vi "Main.vi"() -> ()   [LabVIEW 2021]
doc: "This template is for the Queued Message Handler design pattern.\n\nThe Event Handling Loop generates messages based on user interface actions.\n\nThe Message Handling Loop processes messages generated by the Event Handling Loop, or by other messages. The messages are string values, so new messages can be added easily to the Message Cases case structure in the Message Handling Loop. Each message cluster can also provide an optional value for Message Data, which is a variant that can be converted to whatever message-specific data is required."
uses:
  controls/UI Data.ctl
  Main_VI/Control/login_type.ctl
  controls/test_sequence .ctl
  controls/Get_Set.ctl
  Main_VI/Control/Ini.ctl
  Main_VI/Control/Set_Get.ctl
  controls/FGI.ctl
  support/Message Queue/Enqueue Message (Single).vi
  <vilib>/Utility/error.llb/Error Cluster From Error Code.vi
  <vilib>/ErrorRing/Error Ring.xnode
  support/Message Queue/Message Queue.lvlib
  support/User Event - Stop/User Event - Stop.lvlib
  Main_VI/Control/Vi_selection.ctl
panel:
  out "Test Result":string[][](array[string])
  out "Array":bool[](array[boolean])
  out "element":string[][](array[string])
  out "Elapsed Time (s)":dbl
  out "stop":bool
  out "Update timer":bool
  out "reset timer":bool
  out "Result":bool
  in  "Back Button":bool
  out "Tab Control":enum32{" START ", " HOME ", " TEST "}(tab)
  in  "Uncheck":bool
  in  "Check":bool
  out "FAIL":string
  out "TOTAL":string
  out "PASS":string
  out "?":string
  out "?":string
  out "Test Time":string
  out "Applied 4":string
  out "String Indicator":string
  in  "Start Button":bool
  in  "Main Test Status":i32(listbox)=-1
  in  "Report folder":bool
  in  "Exit":bool
  in  "error in (no error)":errorcluster
  out "Display <Replace Me>":string
  in  "Do Something Else <Replace Me>":bool
  # "REV"
  # "TEST TIME"
  # "BARCODE"
  # "TOTAL"
  # "PASS"
  # "FAIL"
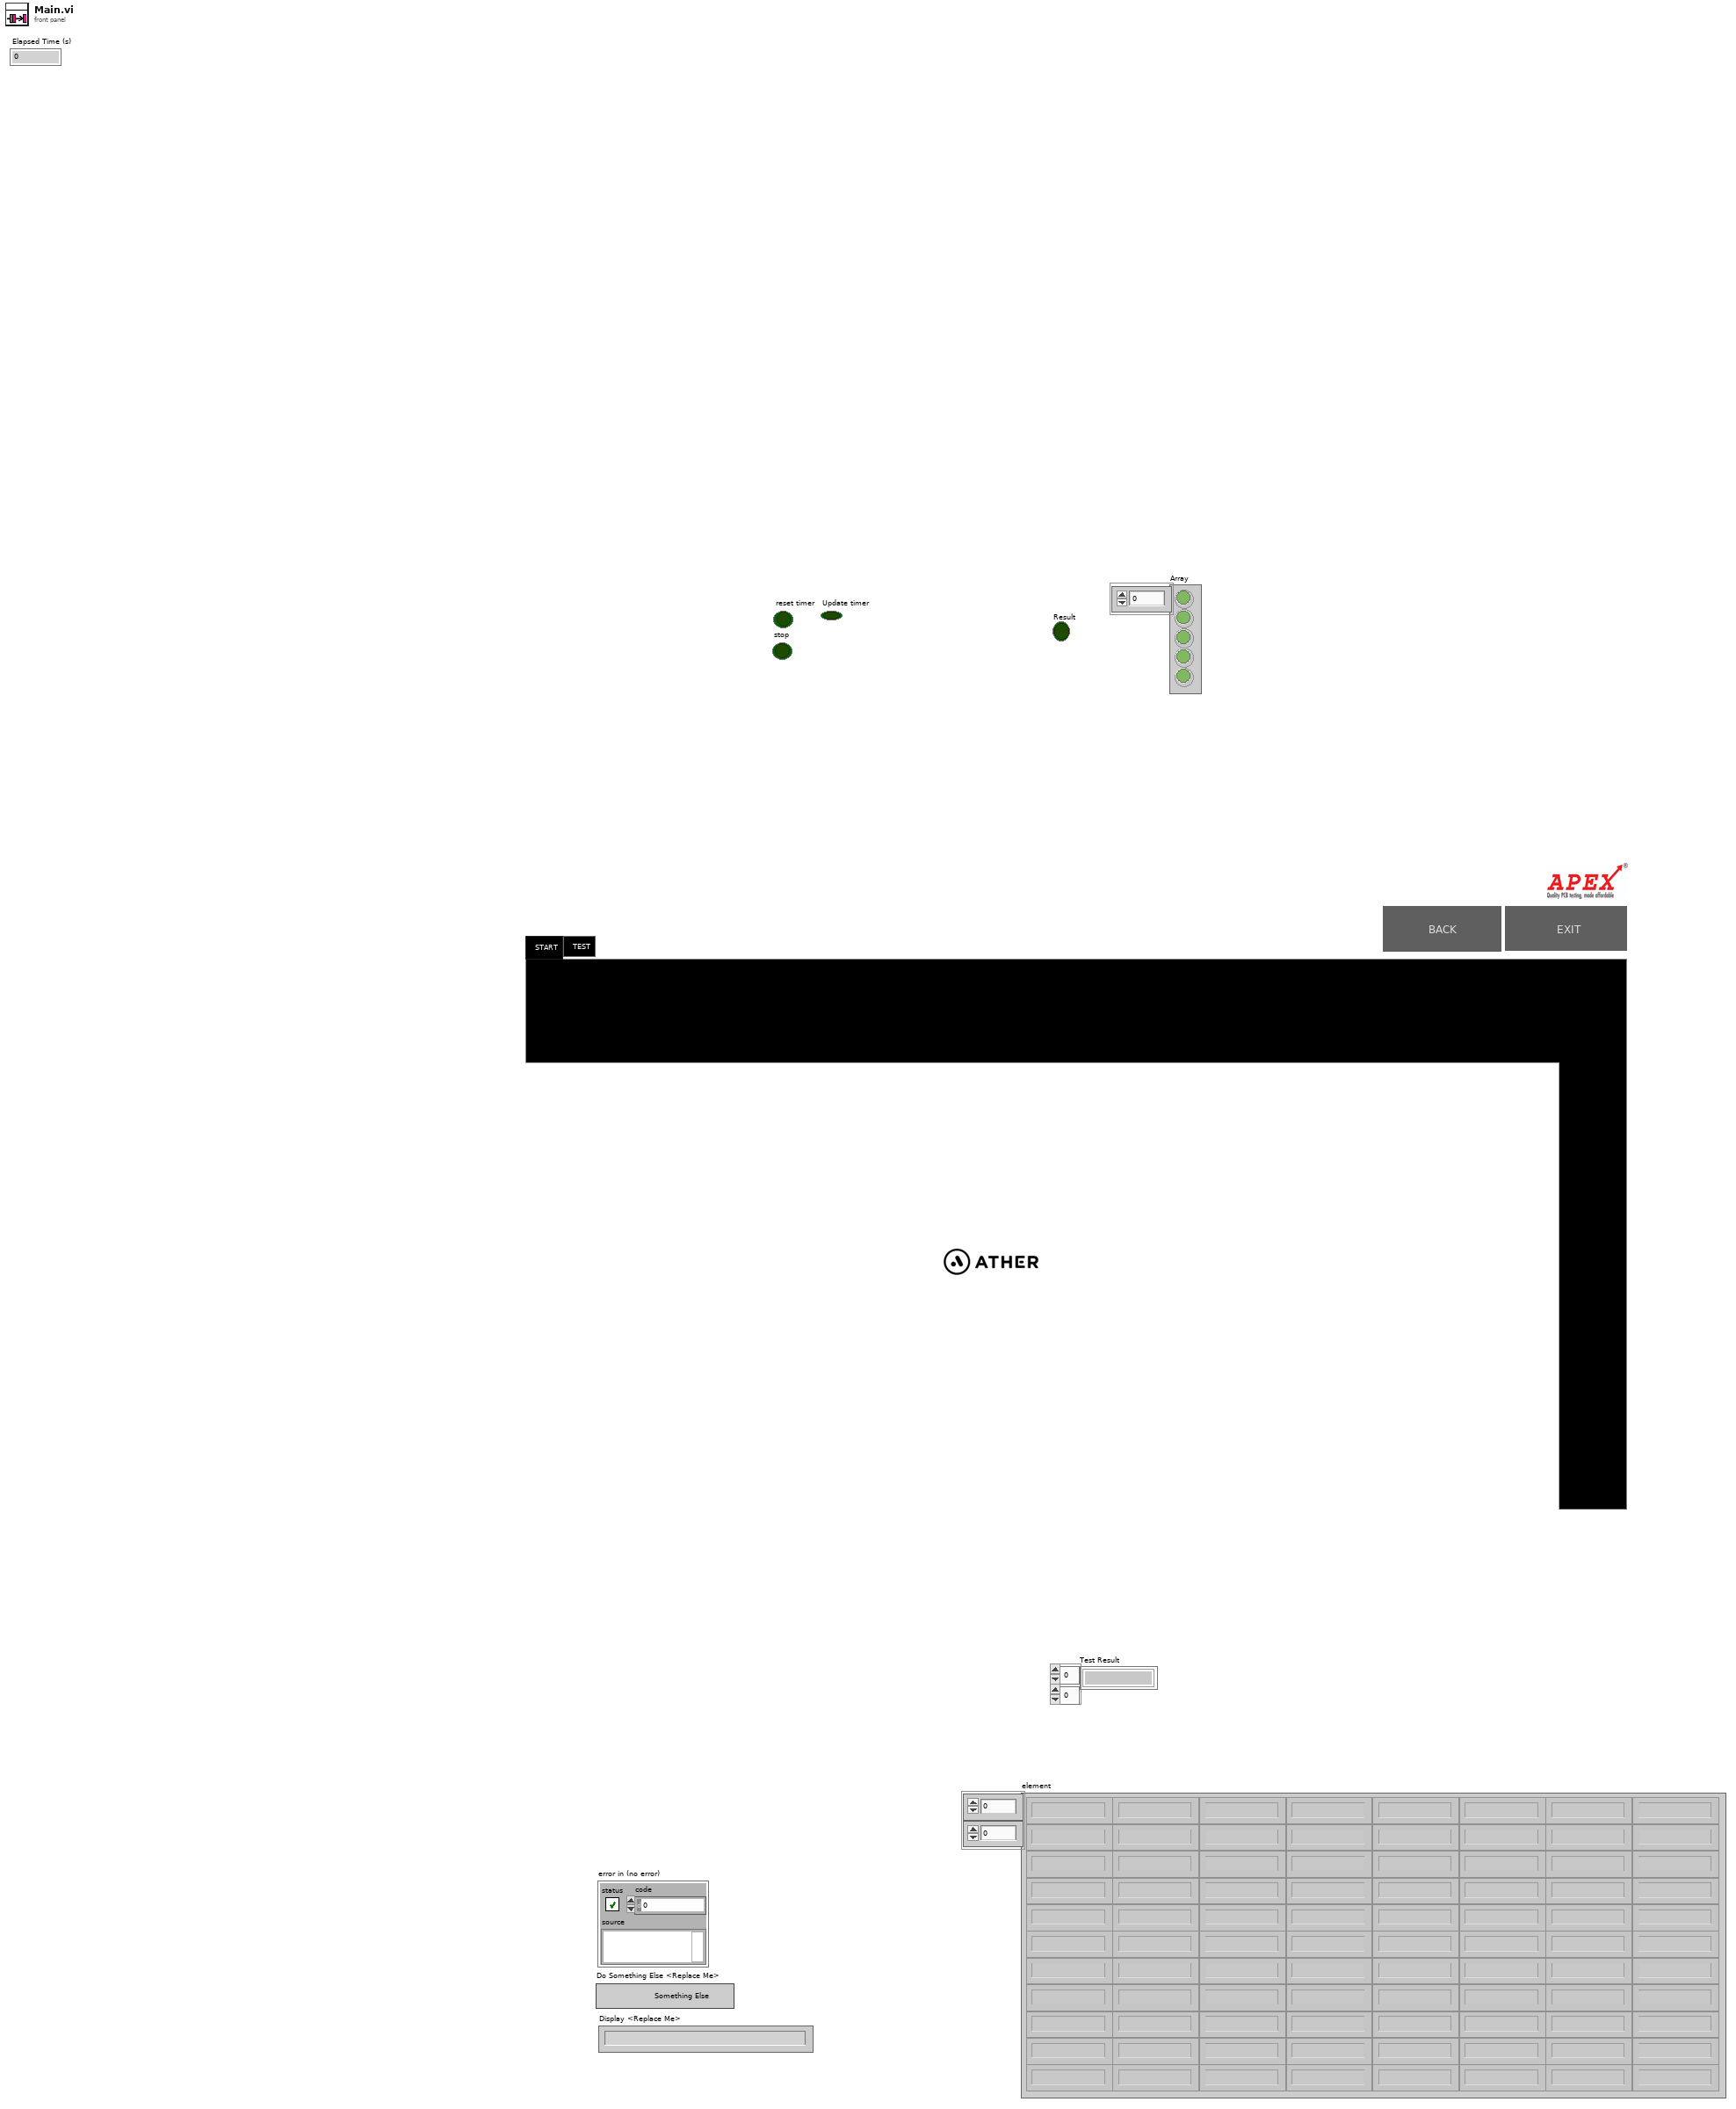
[diagram p1: front panel]
types:
  T1 = typedef "UI Data.ctl" = cluster{"Boolean <Replace Me>":bool, "String <Replace Me>":string, "Numeric <Replace Me>":dbl, "Do Something Ref":refnum<vi>, "Do Something Else Ref":refnum<vi>, "Data Display Ref":refnum<vi>, "Exit Button Ref":refnum<vi>, "Enum":T2, "skip Test  ":bool[]}
  T2 = typedef "login_type.ctl" = enum16{"Operator", "Admin"}
  T3 = typedef "Message Queue.lvlib/All Message Queues.ctl" = cluster{"UI":refnum<queue>}
  T4 = typedef "test_sequence .ctl" = enum16{"Init Devices", "Login", "Option Window", "Idle state", "Check", "Uncheck", "Scan Barcode", "Clear the test Containers", "Init-Pre Test", "Test ", "Result", "Report", "Database", "Update Display", "Confirm Quit", "Error", "Exit"}
  T5 = typedef "LVPoint32TypeDef.ctl" = cluster{"Horizontal":i32, "Vertical":i32}
  T6 = typedef "Ini.ctl" = enum16{"Write", "Read"}
  T7 = enum32{"Invalid", "Standard", "Closed", "Hidden", "Minimized", "Maximized"}
  T8 = typedef "Set_Get.ctl" = enum16{"Set", "Get"}
  T9 = typedef "Vi_selection.ctl" = enum16{"Test Editor", "Option window Vi"}
  T10 = typedef "FGI.ctl" = enum16{"Test Col 1", "Test Col 2"}
  T11 = enum8{"Enabled", "Disabled", "Disabled and Grayed Out"}
  T12 = typedef "Get_Set.ctl" = enum16{"SET", "GET"}
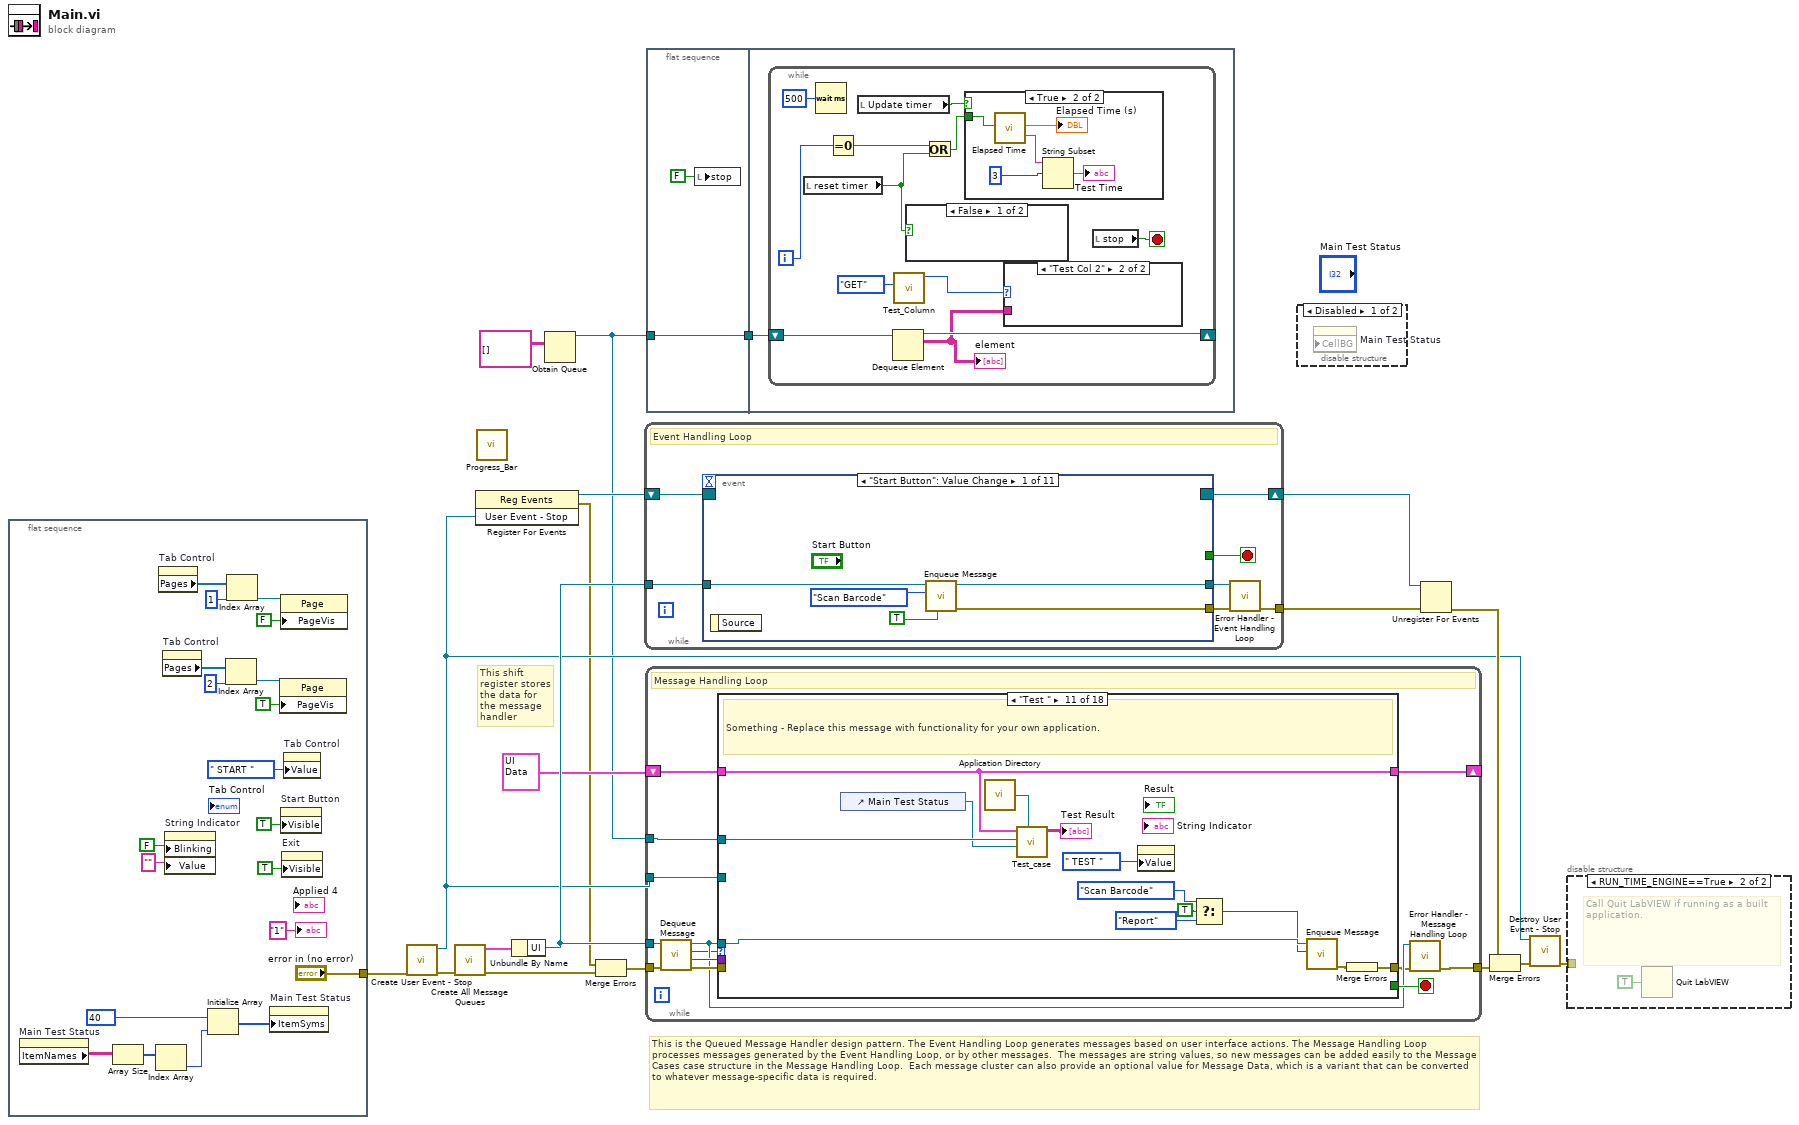
[diagram p0: block diagram]
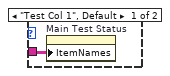
[diagram p3: hidden frame]
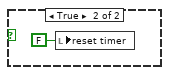
[diagram p4: hidden frame]
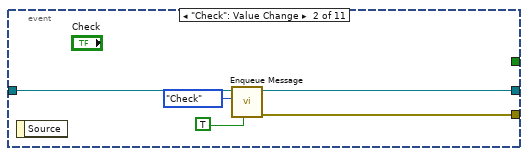
[diagram p7: hidden frame]
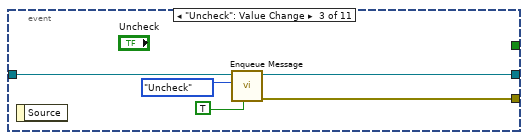
[diagram p8: hidden frame]
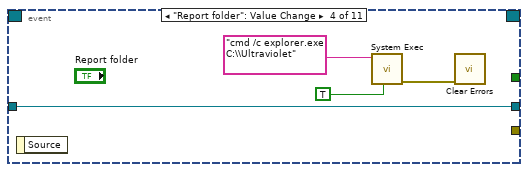
[diagram p9: hidden frame]
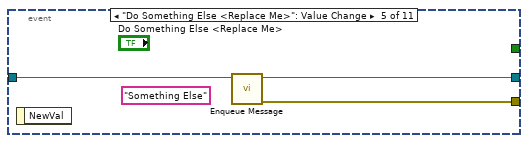
[diagram p10: hidden frame]
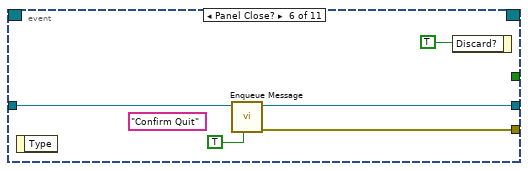
[diagram p11: hidden frame]
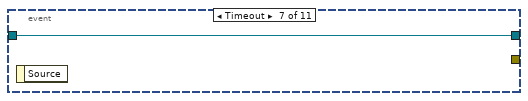
[diagram p12: hidden frame]
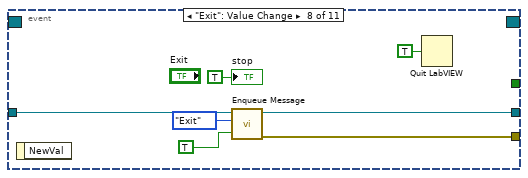
[diagram p13: hidden frame]
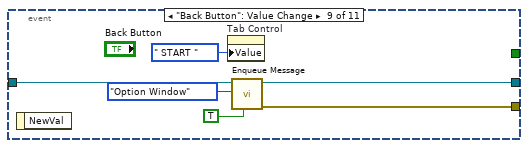
[diagram p14: hidden frame]
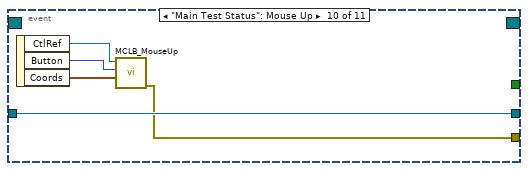
[diagram p15: hidden frame]
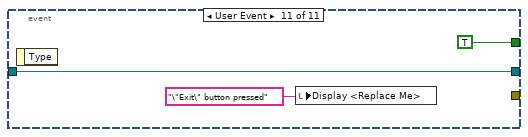
[diagram p16: hidden frame]
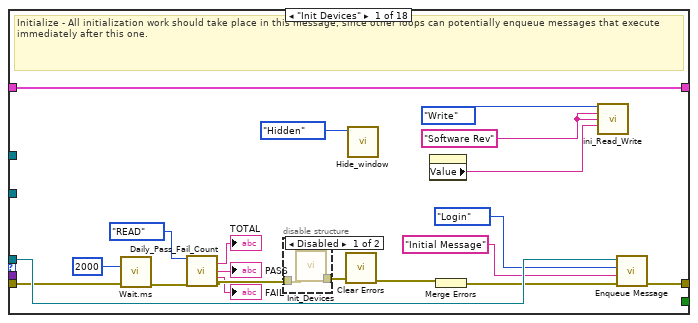
[diagram p17: hidden frame]
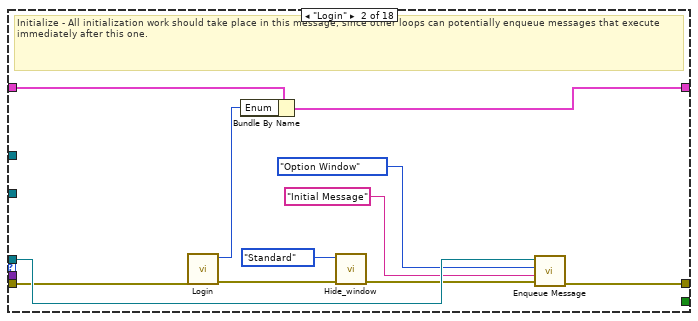
[diagram p19: hidden frame]
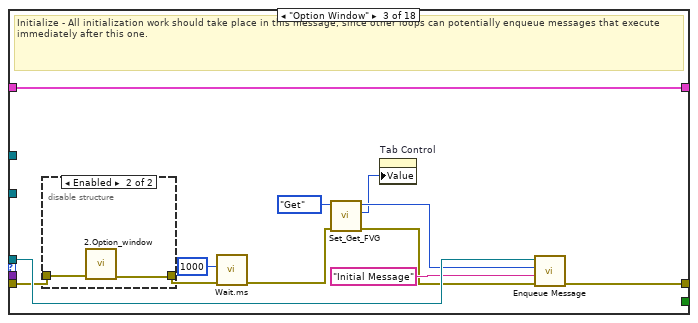
[diagram p20: hidden frame]
diagram:
  # "This is the Queued Message Handler design pattern. The Event Handling Loop generates messages based on user interface actions. The Message Handling Loop processes messages generated by the Event Handling Loop, or by other messages.  The messages are string values, so new messages can be added easily to the Message Cases case structure in the Message Handling Loop.  Each message cluster can also provide an optional value for Message Data, which is a variant that can be converted to whatever message-specific data is required."
  # "This shift register stores the data for the message handler"
  n1 = flat-sequence {
    tunnel: ["error in (no error)"] -> w5
    frame #0 {
      n2 = property on="Main Test Status" class="MCListbox (strict)"() -> ("ItemNames"=w21:string[][])  [unwired: 2 in, 2 out]
      n3 = Array Size(array=w21) -> (size(s)=w22:i32[])
      n4 = Index Array(array=w22) -> (element=w23:i32)  [unwired: 1 in]
      n5 = property on="Tab Control" class="TabCtl (strict)"() -> ("Pages"=w38:refnum<vi>[])  [unwired: 2 in, 2 out]
      n6 = property on="Tab Control" class="TabCtl (strict)"() -> ("Pages"=w32:refnum<vi>[])  [unwired: 2 in, 2 out]
      n7 = property on="String Indicator" class="Str"("Blinking"=FALSE, "Value"="" ("String Indicator")) -> ()  [unwired: 2 in, 2 out]
      n8 = Initialize Array(40, w23) -> (w24:i32[])
      n9 = Index Array(array=w32, index=2) -> (element=w33:refnum<vi>)
      n10 = Index Array(array=w38, index=1) -> (element=w39:refnum<vi>)
      n11 = property on="Main Test Status" class="MCListbox (strict)"("ItemSyms"=w24) -> ()  [unwired: 2 in, 2 out]
      n12 = property class="Page"(reference=w33, "PageVis"=TRUE ("Page Visible")) -> ()  [unwired: 1 in, 2 out]
      n13 = property class="Page"(reference=w39, "PageVis"=FALSE ("Page Visible")) -> ()  [unwired: 1 in, 2 out]
      n14 = property on="Start Button" class="Bool"("Visible"=TRUE) -> ()  [unwired: 2 in, 2 out]
      n15 = property on="Exit" class="Bool"("Visible"=TRUE) -> ()  [unwired: 2 in, 2 out]
      n16 = property on="Tab Control" class="TabCtl (strict)"("Value"=enum32{" START ", " HOME ", " TEST "}." START " ("Tab Control")) -> ()  [unwired: 2 in, 2 out]
      "?" <- "1"
    }
  }
  n17 = call "Create User Event - Stop.vi"("error in (no error)"=w5) -> ("error out"=w15:errorcluster, "User Event - Stop"=w7:refnum<user-event>)  [unwired: 9 in]
  n18 = call "Create All Message Queues.vi"("error in (no error)"=w15) -> ("error out"=w19:errorcluster, "Message Queues out"=w18:T3)  [unwired: 9 in]
  n19 = register-events(w7) -> (reference out=w8:refnum<event-registration>, error out=w4:errorcluster)  [unwired: 2 in]
  n20 = call "Progress_Bar.vi"() -> ()  [unwired: 11 in, 1 out]
  n21 = Unbundle By Name(w18) -> ("UI"=w16:refnum<queue>)
  n22 = Obtain Queue(element data type=string[][] [] ("Test status item names")) -> (queue out=w1:refnum<queue>)  [unwired: 4 in, 2 out]
  n23 = Merge Errors(w4, w19) -> (w6:errorcluster)
  n24 = while {
    tunnel: w16 -> [w46]
    shift-right: [w44] -> w12
    shift-left: w8 -> [w45]
    tunnel: [w40] -> w9
    stop <- w42 stop-if-true
    # "Event Handling Loop"
    n25 = event shown="[0] \"Start Button\": Value Change" {
      selector: w45 -> [_ _ _ _ _ _ _ _ _ _ _]
      dyn-events: [_ _ _ _ _ _ _ _ _ _ _] -> w44
      timeout: _ -> [_ _ _ _ _ _ _ _ _ _ _]
      tunnel: [_ _ _ _ _ _ _ _ _ _ TRUE ("Discard?")] -> w42
      tunnel: w46 -> [w51 w56 w61 w65 w68 w72 w74 w81 w87 w92 w95]
      tunnel: [w49 w54 w59 _ w66 w71 _ w80 w86 w91 _] -> w43
      tunnel: [w50 w55 w60 w65 w67 w70 w74 w79 w85 w92 w95] -> w41
      event "Start Button": Value Change {
        n26 = event-data() -> ()  [unwired: 1 in, 1 out]
        n27 = call-poly "Enqueue Message.vi"("Priority Message? (F)"=TRUE, "Message"=test_sequence_."Scan Barcode", "Message Queue"=w51) -> ("error out"=w49:errorcluster, "dup Message Queue"=w50:refnum<queue>)  [unwired: 7 in]
      }
      event "Check": Value Change {
        n28 = event-data() -> ()  [unwired: 1 in, 1 out]
        n29 = call-poly "Enqueue Message.vi"("Priority Message? (F)"=TRUE, "Message"=test_sequence_."Check", "Message Queue"=w56) -> ("error out"=w54:errorcluster, "dup Message Queue"=w55:refnum<queue>)  [unwired: 7 in]
      }
      event "Uncheck": Value Change {
        n30 = event-data() -> ()  [unwired: 1 in, 1 out]
        n31 = call-poly "Enqueue Message.vi"("Priority Message? (F)"=TRUE, "Message"=test_sequence_."Uncheck", "Message Queue"=w61) -> ("error out"=w59:errorcluster, "dup Message Queue"=w60:refnum<queue>)  [unwired: 7 in]
      }
      event "Report folder": Value Change {
        n32 = event-data() -> ()  [unwired: 1 in, 1 out]
        n33 = call <vilib>:"System Exec.vi"("run minimized? (F)"=TRUE, "command line"="cmd /c explorer.exe C:\\Ultraviolet") -> ("error out"=w62:errorcluster)  [unwired: 6 in, 3 out]
        n34 = call <vilib>:"Clear Errors.vi"("error in (no error)"=w62) -> ()  [unwired: 5 in, 2 out]
      }
      event "Do Something Else <Replace Me>": Value Change {
        (unwired) "Something Else" ("Message")
        n35 = event-data() -> ()  [unwired: 1 in, 1 out]
        n36 = call-poly "Enqueue Message.vi"("Message Queue"=w68) -> ("error out"=w66:errorcluster, "dup Message Queue"=w67:refnum<queue>)  [unwired: 9 in]
      }
      event Panel Close? {
        (unwired) "Confirm Quit" ("Message")
        n37 = event-data() -> ()  [unwired: 1 in, 1 out]
        n38 = call-poly "Enqueue Message.vi"("Priority Message? (F)"=TRUE, "Message Queue"=w72) -> ("error out"=w71:errorcluster, "dup Message Queue"=w70:refnum<queue>)  [unwired: 8 in]
        n39 = event-data("Discard?"=TRUE) -> ()  [unwired: 1 in, 1 out]
      }
      event Timeout {
        n40 = event-data() -> ()  [unwired: 1 in, 1 out]
      }
      event "Exit": Value Change {
        n41 = event-data() -> ()  [unwired: 1 in, 1 out]
        n42 = call-poly "Enqueue Message.vi"("Priority Message? (F)"=TRUE, "Message"=test_sequence_."Exit", "Message Queue"=w81) -> ("error out"=w80:errorcluster, "dup Message Queue"=w79:refnum<queue>)  [unwired: 7 in]
        n43 = Quit LabVIEW(quit? (T)=TRUE) -> ()
        "stop" <- TRUE ("stop")
      }
      event "Back Button": Value Change {
        n44 = event-data() -> ()  [unwired: 1 in, 1 out]
        n45 = property on="Tab Control" class="TabCtl (strict)"("Value"=enum32{" START ", " HOME ", " TEST "}." START " ("Tab Control")) -> ()  [unwired: 2 in, 2 out]
        n46 = call-poly "Enqueue Message.vi"("Priority Message? (F)"=TRUE, "Message"=test_sequence_."Option Window", "Message Queue"=w87) -> ("error out"=w86:errorcluster, "dup Message Queue"=w85:refnum<queue>)  [unwired: 7 in]
      }
      event "Main Test Status": Mouse Up {
        n47 = event-data() -> ("CtlRef"=w88:refnum<vi>, "Button"=w89:u16, "Coords"=w90:T5)  [unwired: 1 in]
        n48 = call "MCLB_MouseUp.vi"("Coords"=w90, "Button"=w89, "CtlRef"=w88) -> ("error out"=w91:errorcluster)  [unwired: 8 in]
      }
      event User Event {
        n49 = event-data() -> ()  [unwired: 1 in, 1 out]
        n50 = local write "Display <Replace Me>"("\"Exit\" button pressed" ("VI Stopped")) -> ()
      }
    }
    n51 = call "Error Handler - Event Handling Loop.vi"("error in (no error)"=w43, "Message Queue"=w41) -> ("dup error in"=w40:errorcluster)  [unwired: 8 in, 1 out]
  }
  n52 = while {
    tunnel: w16 -> [w101]
    shift-right: [w107] -> _
    shift-left: T1 {"Boolean <Replace Me>"=FALSE, "String <Replace Me>"="", "Numeric <Replace Me>"=0.0, "Do Something Ref"=refnum, "Do Something Else Ref"=refnum, "Data Display Ref"=refnum, "Exit Button Ref"=refnum, "Enum"=enum."Admin", "skip Test  "=[]} ("Data Cluster") -> [w108]
    tunnel: w7 -> [w105]
    tunnel: w6 -> [w104]
    tunnel: [w99] -> w17
    tunnel: w1 -> [w96]
    stop <- w106 stop-if-true
    # "Message Handling Loop"
    n53 = call "Dequeue Message.vi"("error in (no error)"=w104, "Message Queue"=w101) -> ("error out"=w103:errorcluster, "Message Data"=w102:variant, "Message"=w97:T4, "dup Message Queue"=w100:refnum<queue>)  [unwired: 6 in]
    n54 = case "Message Cases" shown="\"Test \"" w97 {
      selector: w97 -> [_ _ _ _ _ _ _ _ _ _ _ _ _ _ _ _ _ w344]
      tunnel: w100 -> [w127 w141 w153 _ _ w179 w189 w219 w245 w252 w272 w290 w302 w312 _ w327 w343 _]
      tunnel: w103 -> [w111 w138 w150 w165 w177 w181 w191 w213 w242 w256 _ w288 w298 w309 w324 w331 w336 _]
      tunnel: [w128 w142 w154 w166 w177 w180 w190 w221 w247 w260 w274 w292 w304 w314 w318 w329 w339 w345] -> w98
      tunnel: w108 -> [w125 w137 w151 w167 w176 w187 w197 w200 w248 w261 w265 w293 w305 w315 w323 w330 w342 w346]
      tunnel: [w125 w136 w151 w167 w176 w187 w197 w198 w248 w261 w265 w293 w305 w315 w323 w330 w342 w346] -> w107
      tunnel: [_ _ _ _ _ _ _ _ _ _ _ _ _ _ _ _ TRUE _] -> w106
      tunnel: w102 -> [_ _ _ w164 _ _ _ _ _ _ _ _ _ _ w322 _ w333 _]
      tunnel: w105 -> [_ _ _ _ _ _ _ _ _ _ _ _ _ _ _ _ w338 _]
      tunnel: w96 -> [_ _ _ _ _ _ _ _ _ _ w266 _ _ _ _ _ _ _]
      frame "Init Devices" {
        w118 = "Software Rev" ("Write Section")
        # "Initialize - All initialization work should take place in this message, since other loops can potentially enqueue messages that execute immediately after this one."
        n55 = call "Wait.ms.vi"("error in"=w111, "milliseconds to wait"=u32 2000) -> ("error out"=w110:errorcluster)  [unwired: 9 in]
        n56 = call "Daily_Pass_Fail_Count.vi"("Action"=enum16{"READ", "WRITE"}."READ", "error in"=w110) -> ("TOTAL"=→"TOTAL":string, "PASS"=→"PASS":string, "FAIL"=→"FAIL":string, "error out"=w116:errorcluster)  [unwired: 8 in, 2 out]
        n57 = disable-structure shown="Disabled" {
          disable-tunnel: [w130 w131] -> w124
          disable-tunnel: w116 -> [w129 w131]
          frame Disabled {
            n58 = call "Init_Devices.vi"("error in"=w129) -> ("error out"=w130:errorcluster)  [unwired: 9 in, 1 out]
          }
          frame Enabled {
          }
        }
        n59 = call <vilib>:"Clear Errors.vi"("error in (no error)"=w124) -> ("error out"=w122:errorcluster)  [unwired: 5 in, 1 out]
        n60 = call "Hide_window.vi"("State"=T7."Hidden") -> ()  [unwired: 10 in, 1 out]
        n61 = property class="Str"() -> ("Value"=w117:string)  [unwired: 2 in, 2 out]
        n62 = Merge Errors(w122) -> (w123:errorcluster)
        n63 = call "ini_Read_Write.vi"(0:Ini."Write", "Write Section"=w118, "Write key"=w118, "Write"=w117) -> ()  [unwired: 10 in, 2 out]
        n64 = call-poly "Enqueue Message.vi"("error in (no error)"=w123, "Message Data"="Initial Message" ("Initial Message"), "Message"=test_sequence_."Login", "Message Queue"=w127) -> ("error out"=w128:errorcluster)  [unwired: 6 in, 1 out]
      }
      frame "Login" {
        # "Initialize - All initialization work should take place in this message, since other loops can potentially enqueue messages that execute immediately after this one."
        n65 = call "Login.vi"("error in (no error) 3"=w138) -> ("error in (no error) 4"=w134:errorcluster, "Enum"=w132:T2)  [unwired: 9 in]
        n66 = Bundle By Name(cluster=w137, "Enum"=w132) -> (w136:T1)
        n67 = call "Hide_window.vi"("error in (no error)"=w134, "State"=T7."Standard") -> ("error out"=w133:errorcluster)  [unwired: 9 in]
        n68 = call-poly "Enqueue Message.vi"("error in (no error)"=w133, "Message Data"="Initial Message" ("Initial Message"), "Message"=test_sequence_."Option Window", "Message Queue"=w141) -> ("error out"=w142:errorcluster)  [unwired: 6 in, 1 out]
      }
      frame "Option Window" {
        # "Initialize - All initialization work should take place in this message, since other loops can potentially enqueue messages that execute immediately after this one."
        n69 = disable-structure shown="Enabled" {
          disable-tunnel: w150 -> [w157 w159]
          disable-tunnel: [w156 w158] -> w149
          frame Disabled {
            n70 = call "3.Open_Vi.vi"("error in (no error)"=w157, "VI Selection"=Vi_selection."Option window Vi") -> ("error out"=w156:errorcluster)  [unwired: 9 in]
          }
          frame Enabled {
            n71 = call "2.Option_window.vi"("error in (no error) 2"=w159) -> ("error in (no error) 3"=w158:errorcluster)  [unwired: 10 in]
          }
        }
        n72 = call "Wait.ms.vi"("error in"=w149, "milliseconds to wait"=u32 1000) -> ("error out"=w145:errorcluster)  [unwired: 9 in]
        n73 = call "Set_Get_FVG.vi"("error out"=w145, "Enum"=Set_Get."Get") -> ("error out 2"=w144:errorcluster, "Tab Control 2"=w143:enum32{" START ", " HOME ", " TEST "}, "Message 2"=w146:T4)  [unwired: 7 in]
        n74 = property on="Tab Control" class="TabCtl (strict)"("Value"=w143) -> ()  [unwired: 2 in, 2 out]
        n75 = call-poly "Enqueue Message.vi"("error in (no error)"=w144, "Message Data"="Initial Message" ("Initial Message"), "Message"=w146, "Message Queue"=w153) -> ("error out"=w154:errorcluster)  [unwired: 6 in, 1 out]
      }
      frame "Update Display" {
        w161 = T11."Enabled" ("Disabled")
        # "Update Display - Convert the message data to a string to display in the Data Display indicator."
        n76 = disable-structure shown="Enabled" {
          disable-tunnel: w165 -> [w172 w173]
          disable-tunnel: w164 -> [w171 _]
          disable-tunnel: [w169 w173] -> w160
          frame Disabled {
            n77 = Variant To Data(error in=w172, type="", Variant=w171) -> (data=→"Display <Replace Me>":string, error out=w169:errorcluster)
          }
          frame Enabled {
          }
        }
        n78 = property class="Str"("Value"="") -> ()  [unwired: 2 in, 2 out]
        n79 = property on="Applied 4" class="Str"("Value"="" ("Applied 4")) -> ()  [unwired: 2 in, 2 out]
        n80 = property on="Start Button" class="Bool"("DisabledEnum"=w161) -> ()  [unwired: 2 in, 2 out]
        n81 = property on="Back Button" class="Bool"("DisabledEnum"=w161) -> ()  [unwired: 2 in, 2 out]
        n82 = property on="Exit" class="Bool"("DisabledEnum"=w161) -> ()  [unwired: 2 in, 2 out]
        n83 = Merge Errors(w160) -> (w166:errorcluster)
      }
      frame "Idle state" {
        w174 = T11."Enabled" ("Disabled")
        n84 = property on="Applied 4" class="Str"("Value"="" ("Applied 4")) -> ()  [unwired: 2 in, 2 out]
        n85 = property on="Start Button" class="Bool"("DisabledEnum"=w174) -> ()  [unwired: 2 in, 2 out]
        n86 = property on="Back Button" class="Bool"("DisabledEnum"=w174) -> ()  [unwired: 2 in, 2 out]
        n87 = property on="Exit" class="Bool"("DisabledEnum"=w174) -> ()  [unwired: 2 in, 2 out]
      }
      frame "Uncheck" {
        n88 = property on="Main Test Status" class="MCListbox (strict)"() -> ("ItemNames"=w185:string[][])  [unwired: 2 in, 2 out]
        n89 = Array Size(array=w185) -> (size(s)=w184:i32[])
        n90 = Index Array(array=w184) -> (element=w183:i32)  [unwired: 1 in]
        n91 = Initialize Array(39, w183) -> (w182:i32[])
        n92 = property on="Main Test Status" class="MCListbox (strict)"("ItemSyms"=w182) -> ()  [unwired: 2 in, 2 out]
        n93 = call-poly "Enqueue Message.vi"("error in (no error)"=w181, "Message"=test_sequence_."Idle state", "Message Queue"=w179) -> ("error out"=w180:errorcluster)  [unwired: 7 in, 1 out]
      }
      frame "Check" {
        n94 = property on="Main Test Status" class="MCListbox (strict)"() -> ("ItemNames"=w195:string[][])  [unwired: 2 in, 2 out]
        n95 = Array Size(array=w195) -> (size(s)=w194:i32[])
        n96 = Index Array(array=w194) -> (element=w193:i32)  [unwired: 1 in]
        n97 = Initialize Array(40, w193) -> (w192:i32[])
        n98 = property on="Main Test Status" class="MCListbox (strict)"("ItemSyms"=w192) -> ()  [unwired: 2 in, 2 out]
        n99 = call-poly "Enqueue Message.vi"("error in (no error)"=w191, "Message"=test_sequence_."Idle state", "Message Queue"=w189) -> ("error out"=w190:errorcluster)  [unwired: 7 in, 1 out]
      }
      frame "Scan Barcode" {
        # "Something - Replace this message with functionality for your own application."
        n100 = property class="Str"(error in=w213, "Value"="") -> (error out=w212:errorcluster)  [unwired: 1 in, 1 out]
        n101 = call "MSG display box two buttons.vi"("error in"=w212, "input string"="Place the DUT , Close The Top Gate and Press OK or Prees ENTER key\n\nThen DO NOT TOUCH FIXTURE") -> ("error out"=w208:errorcluster, "Panel close"=w210:bool)  [unwired: 7 in, 1 out]
        n102 = property on="Tab Control" class="TabCtl (strict)"("Value"=enum32{" START ", " HOME ", " TEST "}." TEST " ("Tab Control")) -> ()  [unwired: 2 in, 2 out]
        n103 = case shown="False" w210 {
          tunnel: w208 -> [w226 w239]
          tunnel: [w228 w239] -> w203
          tunnel: [w227 TRUE ("Time has Elapsed")] -> w211
          frame False {
            n104 = case shown="False" FALSE {
              tunnel: [w231 _] -> w228
              tunnel: [w230 FALSE ("Time has Elapsed")] -> w227
              tunnel: w226 -> [w229 _]
              frame False {
                n105 = disable-structure shown="Disabled" {
                  disable-tunnel: [w235 _] -> w231
                  disable-tunnel: [w234 _] -> w230
                  disable-tunnel: w229 -> [w232 _]
                  frame Disabled {
                    n106 = call "Barcode user prompt.vi"("error in"=w232) -> ("error out"=w235:errorcluster, "Time has Elapsed"=w234:bool, "BARCODE"=→"?":string)  [unwired: 8 in]
                  }
                  frame Enabled {
                  }
                }
              }
              frame True {
                n107 = One Button Dialog(message="              INTERLOCK OPEN \nClose the top gate and press start") -> ()  [unwired: 1 in, 1 out]
              }
            }
          }
          frame True {
          }
        }
        n108 = property on="Main Test Status" class="MCListbox (strict)"() -> ("ItemSyms"=w201:i32[])  [unwired: 2 in, 2 out]
        n109 = property on="Applied 4" class="Str"(error in=w208, "Value"="SCANNING BARCODE" ("Applied 4")) -> ()  [unwired: 1 in, 2 out]
        n110 = for {
          tunnel: w201 -> [w224] mode=indexing
          tunnel: [w222] -> w199 mode=indexing
          n111 = Equal?(x=w224, y=40) -> (x = y?=w222:bool)
        }
        "Array" <- w199
        n112 = Compound Arithmetic op=OR(w211, w210) -> (w209:bool)
        n113 = Bundle By Name(cluster=w200, "skip Test"=w199) -> (w198:T1)
        n114 = Select(t=test_sequence_."Idle state", s=w209, f=test_sequence_."Clear the test Containers" ("Message")) -> (s? t:f=w215:T4)
        n115 = call "Start_Time.vi"("error in (no error)"=w203) -> ("error in (no error) 3"=w204:errorcluster)  [unwired: 10 in]
        n116 = call-poly "Enqueue Message.vi"("error in (no error)"=w204, "Message"=w215, "Message Queue"=w219) -> ("error out"=w220:errorcluster)  [unwired: 7 in, 1 out]
        n117 = property on="String Indicator" class="Str"("Blinking"=FALSE, "Value"="" ("String Indicator")) -> ()  [unwired: 2 in, 2 out]
        n118 = Merge Errors(w220) -> (w221:errorcluster)
      }
      frame "Clear the test Containers" {
        w241 = TRUE ("reset timer")
        w240 = T11."Disabled and Grayed Out" ("Disabled")
        # "Something - Replace this message with functionality for your own application."
        n119 = property on="Tab Control" class="TabCtl (strict)"("Value"=enum32{" START ", " HOME ", " TEST "}." TEST " ("Tab Control")) -> ()  [unwired: 2 in, 2 out]
        n120 = call-poly "Enqueue Message.vi"("error in (no error)"=w242, "Message"=test_sequence_."Init-Pre Test", "Message Queue"=w245) -> ("error out"=w246:errorcluster)  [unwired: 7 in, 1 out]
        n121 = property on="Start Button" class="Bool"("DisabledEnum"=w240) -> ()  [unwired: 2 in, 2 out]
        n122 = property on="Exit" class="Bool"("DisabledEnum"=w240) -> ()  [unwired: 2 in, 2 out]
        n123 = property on="Back Button" class="Bool"("DisabledEnum"=w240) -> ()  [unwired: 2 in, 2 out]
        n124 = Merge Errors(w246) -> (w247:errorcluster)
        "reset timer" <- w241
        "Update timer" <- w241
      }
      frame "Init-Pre Test" {
        # "Something - Replace this message with functionality for your own application."
        n125 = property on="Main Test Status" class="MCListbox (strict)"("ItemNames"=string[][] [] ("Item Names")) -> ()  [unwired: 2 in, 2 out]
        n126 = property on="Applied 4" class="Str"(error in=w256, "Value"="" ("Applied 4")) -> (error out=w251:errorcluster)  [unwired: 1 in, 1 out]
        n127 = call "Test_Column.vi"("Enum"=FGI."Test Col 1") -> ()  [unwired: 10 in, 1 out]
        n128 = call-poly "Enqueue Message.vi"("error in (no error)"=w251, "Message"=test_sequence_."Test ", "Message Queue"=w252) -> ("error out"=w259:errorcluster)  [unwired: 7 in, 1 out]
        n129 = property on="String Indicator" class="Str"(error in=w256, "Blinking"=TRUE, "Value"="TEST IN PROGRESS DO NOT TOUCH FIXTURE" ("String Indicator")) -> ()  [unwired: 1 in, 2 out]
        n130 = Merge Errors(w259) -> (w260:errorcluster)
        n131 = property on="Tab Control" class="TabCtl (strict)"("Value"=enum32{" START ", " HOME ", " TEST "}." TEST " ("Tab Control")) -> ()  [unwired: 2 in, 2 out]
      }
      frame "Test " {
        # "Something - Replace this message with functionality for your own application."
        n132 = control-ref of="Main Test Status"() -> (w264:refnum<vi>)
        n133 = call <vilib>:"Application Directory.vi"() -> ("Application Directory"=w262:path)
        n134 = call "Test_case.vi"("base path"=w262, "Main Test Status"=w264, "queue out"=w266, "Data Cluster"=w265) -> ("Result"=→"Test Result":string[][])  [unwired: 7 in]
        n135 = property on="Tab Control" class="TabCtl (strict)"("Value"=enum32{" START ", " HOME ", " TEST "}." TEST " ("Tab Control")) -> ()  [unwired: 2 in, 2 out]
        n136 = Select(t=test_sequence_."Scan Barcode", s=TRUE, f=test_sequence_."Report" ("Message")) -> (s? t:f=w271:T4)
        n137 = call-poly "Enqueue Message.vi"("Message"=w271, "Message Queue"=w272) -> ("error out"=w273:errorcluster)  [unwired: 8 in, 1 out]
        n138 = Merge Errors(w273) -> (w274:errorcluster)
      }
      frame "Result" {
        w278 = T11."Enabled" ("Disabled")
        # "Something - Replace this message with functionality for your own application."
        n139 = property on="Result" class="Bool (strict)"() -> ("Value"=w283:bool)  [unwired: 2 in, 2 out]
        n140 = call "Update_Result.vi"("error in (no error) 2"=w288, "Boolean"=w283) -> ("error in (no error) 3"=w286:errorcluster, "FAIL"=w275:string, "PASS"=w276:string, "TOTAL"=w277:string)  [unwired: 6 in]
        n141 = property on="Tab Control" class="TabCtl (strict)"("Value"=enum32{" START ", " HOME ", " TEST "}." TEST " ("Tab Control")) -> ()  [unwired: 2 in, 2 out]
        n142 = local write "TOTAL"(w277) -> ()
        n143 = local write "PASS"(w276) -> ()
        n144 = local write "FAIL"(w275) -> ()
        n145 = disable-structure shown="Disabled" {
          disable-tunnel: w286 -> [w296 _]
          disable-tunnel: [w295 _] -> w285
          frame Disabled {
            n146 = local read "Test Time"() -> (w294:string)
            n147 = call "Test_Time_Update.vi"("error in (no error) 2"=w296, "Write"=w294) -> ("error in (no error) 3"=w295:errorcluster)  [unwired: 9 in]
          }
          frame Enabled {
          }
        }
        n148 = property on="Back Button" class="Bool"("DisabledEnum"=w278) -> ()  [unwired: 2 in, 2 out]
        n149 = property on="Start Button" class="Bool"("DisabledEnum"=w278) -> ()  [unwired: 2 in, 2 out]
        n150 = property on="Exit" class="Bool"("DisabledEnum"=w278) -> ()  [unwired: 2 in, 2 out]
        n151 = property on="Applied 4" class="Str"("Value"="" ("Applied 4")) -> ()  [unwired: 2 in, 2 out]
        n152 = property on="String Indicator" class="Str"("Blinking"=FALSE, "Value"="" ("String Indicator")) -> ()  [unwired: 2 in, 2 out]
        n153 = property class="Str"("Value"="") -> ()  [unwired: 2 in, 2 out]
        n154 = call-poly "Enqueue Message.vi"("error in (no error)"=w285, "Message"=test_sequence_."Idle state", "Message Queue"=w290) -> ("error out"=w291:errorcluster)  [unwired: 7 in, 1 out]
        n155 = Merge Errors(w291) -> (w292:errorcluster)
        n156 = local write "Update timer"(FALSE ("Update timer")) -> ()
      }
      frame "Report" {
        # "Something - Replace this message with functionality for your own application."
        n157 = property on="Test Result" class="Arr (strict)"() -> ("Value"=w297:string[][])  [unwired: 2 in, 2 out]
        n158 = property on="Result" class="Bool (strict)"() -> ("Value"=w300:bool)  [unwired: 2 in, 2 out]
        n159 = call "CSV_REPORT.vi"(5:"Result"=w300, 8:"Result"=w297) -> ()  [unwired: 26 in]
        n160 = property on="Tab Control" class="TabCtl (strict)"("Value"=enum32{" START ", " HOME ", " TEST "}." TEST " ("Tab Control")) -> ()  [unwired: 2 in, 2 out]
        n161 = call-poly "Enqueue Message.vi"("error in (no error)"=w298, "Message"=test_sequence_."Idle state", "Message Queue"=w302) -> ("error out"=w303:errorcluster)  [unwired: 7 in, 1 out]
        n162 = Merge Errors(w303) -> (w304:errorcluster)
      }
      frame "Database" {
        # "Something - Replace this message with functionality for your own application."
        n163 = property on="Result" class="Bool (strict)"() -> ("Value"=w306:bool)  [unwired: 2 in, 2 out]
        n164 = call "IMES.vi"("Boolean"=w306, "error in (no error)"=w309) -> ("error out"=w307:errorcluster)  [unwired: 17 in]
        n165 = flat-sequence {
          tunnel: [w317] -> w308
          tunnel: w307 -> [w317]
          tunnel: w306 -> [w316]
          frame #0 {
            n166 = call "PASS_FAIL_Prompt.vi"("Result"=w316) -> ()  [unwired: 11 in]
          }
        }
        n167 = call-poly "Enqueue Message.vi"("error in (no error)"=w308, "Message"=test_sequence_."Scan Barcode", "Message Queue"=w312) -> ("error out"=w313:errorcluster)  [unwired: 7 in, 1 out]
        n168 = property on="Tab Control" class="TabCtl (strict)"("Value"=enum32{" START ", " HOME ", " TEST "}." TEST " ("Tab Control")) -> ()  [unwired: 2 in, 2 out]
        n169 = Merge Errors(w313) -> (w314:errorcluster)
      }
      frame "Error" {
        # "#CodeRecommended - If you ever change the name of this \"Error\" message, you'll need to update the name in the Check Loop Error.vi as well."
        # "#CodeRecommended - Consider creating a system for logging errors in some way. These errors are for notification purposes only. Handling of specific errors should be performed in the message frames that generated the error."
        # "Error - Display an error dialog. This message is sent by the \"Error Handler\" VIs at the end of other loops in this application."
        n170 = Variant To Data(error in=w324, type=errorcluster {"status"=FALSE, "code"=0, "source"=""} ("error constant"), Variant=w322) -> (data=w320:errorcluster, error out=w319:errorcluster)
        n171 = call <vilib>:"Simple Error Handler.vi"("error in (no error)"=w320) -> ()  [unwired: 4 in, 5 out]
        n172 = Merge Errors(w319) -> (w318:errorcluster)
      }
      frame "Confirm Quit" {
        # "#CodeNeeded - If you want to provide an \"Are you sure\" dialog (or some other notification) before the application exits, place that code here. This message is typically sent from a Panel Close? event."
        # "Confirm Quit - Message that can confirm whether or not the user wants to exit the application."
        n173 = call-poly "Enqueue Message.vi"("Priority Message? (F)"=TRUE, "error in (no error)"=w331, "Message"=test_sequence_."Option Window", "Message Queue"=w327) -> ("error out"=w328:errorcluster)  [unwired: 6 in, 1 out]
        n174 = Merge Errors(w328) -> (w329:errorcluster)
      }
      frame "Exit" {
        # "Exit - Exit the application."
        n175 = Variant To Data(type=errorcluster {"status"=FALSE, "code"=0, "source"=""} ("error constant"), Variant=w333) -> (data=w334:errorcluster)  [unwired: 1 in, 1 out]
        n176 = call <vilib>:"Simple Error Handler.vi"("error in (no error)"=w334) -> ()  [unwired: 4 in, 5 out]
        n177 = local write "stop"(TRUE ("stop")) -> ()
        n178 = Release Queue(queue=w343, error in (no error)=w336) -> (error out=w340:errorcluster)  [unwired: 1 in, 2 out]
        n179 = call "Fire User Event - Stop.vi"("User Event - Stop"=w338) -> ("error out"=w337:errorcluster)  [unwired: 10 in]
        n180 = Merge Errors(w337, w340) -> (w339:errorcluster)
      }
      frame Default {
        # "'Default' case only runs if there is a message that isn't defined in any of the other cases.  Output a programming error."
        n181 = xnode "Error Ring"("parameter 0"=w344) -> ("error out"=w345:errorcluster)
      }
    }
    n182 = call "Error Handler - Message Handling Loop.vi"("error in (no error)"=w98, "Message Queue"=w100) -> ("dup error in"=w99:errorcluster)  [unwired: 8 in, 1 out]
  }
  n183 = flat-sequence {
    tunnel: w1 -> [w354]
    tunnel: [w354] -> w2
    tunnel: w2 -> [w356]
    frame #0 {
      n184 = local write "stop"(FALSE ("stop")) -> ()
    }
    frame #1 {
      n185 = while {
        shift-right: [w360] -> _
        shift-left: w356 -> [w361]
        i -> [w368]
        stop <- w366 stop-if-true
        n186 = local read "reset timer"() -> (w362:bool)
        n187 = Wait (ms)(milliseconds to wait=u32 500) -> ()  [unwired: 1 out]
        n188 = Equal To 0?(x=w368) -> (x = 0?=w365:bool)
        n189 = local read "Update timer"() -> (w363:bool)
        n190 = Dequeue Element(queue=w361) -> (queue out=w360:refnum<queue>, element=w359:string[][])  [unwired: 2 in, 2 out]
        "element" <- w359
        n191 = call "Test_Column.vi"("Enum"=Get_Set."GET") -> ("Enum"=w357:T10)  [unwired: 10 in]
        n192 = case shown="False" w362 {
          frame False {
          }
          frame True {
            n193 = local write "reset timer"(FALSE ("reset timer")) -> ()
          }
        }
        n194 = Or(x=w365, y=w362) -> (x .or. y?=w364:bool)
        n195 = case shown="True" w363 {
          tunnel: w364 -> [_ w373]
          frame False {
          }
          frame True {
            n196 = call "Elapsed Time"("Reset"=w373) -> ("Elapsed Time (s)"=→"Elapsed Time (s)":dbl, "Elapsed Time Text"=w374:string)  [unwired: 11 in, 6 out]
            n197 = String Subset(string=w374, offset (0)=3) -> (substring=→"Test Time":string)  [unwired: 1 in]
          }
        }
        n198 = case shown="\"Test Col 2\"" w357 {
          tunnel: w359 -> [w369 _]
          frame "Test Col 1", Default {
            n199 = property on="Main Test Status" class="MCListbox (strict)"("ItemNames"=w369) -> ()  [unwired: 2 in, 2 out]
          }
          frame "Test Col 2" {
          }
        }
        n200 = local read "stop"() -> (w366:bool)
      }
    }
  }
  n201 = disable-structure shown="Disabled" {
    frame Disabled {
      n202 = property on="Main Test Status" class="MCListbox (strict)" props=["CellBG"]() -> ()  [unwired: 3 in, 2 out]
    }
    frame Enabled {
    }
  }
  n203 = Unregister For Events(event registration refnum=w12, error in=w9) -> (error out=w13:errorcluster)
  n204 = Merge Errors(w13, w17) -> (w14:errorcluster)
  n205 = call "Destroy User Event - Stop.vi"("error in (no error)"=w14, "User Event - Stop"=w7) -> ("error out"=w10:errorcluster)  [unwired: 9 in]
  n206 = disable-structure shown="RUN_TIME_ENGINE==True" {
    disable-tunnel: w10 -> [_ _]
    frame condition #0 (active) {
    }
    frame condition #1 {
      # "Call Quit LabVIEW if running as a built application."
      n207 = Quit LabVIEW(quit? (T)=TRUE) -> ()
    }
  }
